vi "Update MC Listbox vColumn headers.vi"(0 "Multicolumn Listbox Ref":refnum<vi>, 1 "Interpret as Unicode (T)":bool=TRUE, 5 "Column Headers[]":string[](array[string]), 7 "Row Headers[]":string[](array[string]), 11 "Error in":errorcluster) -> (4 "Multicolumn Listbox Ref":refnum<vi>, 15 "error out":errorcluster)   [LabVIEW 2019, in "Language Selection.lvlib"]
doc: "Uses \"Column Header[]\" and \"Row Headers[]\" input arrays to translate a headers of a MulticolumnListbox control.\n- - -\nCopyright (c) 2026, Merecs Engineering GmbH"
uses:
  Language Selection.lvlib
panel:
  # "Connector Pane"
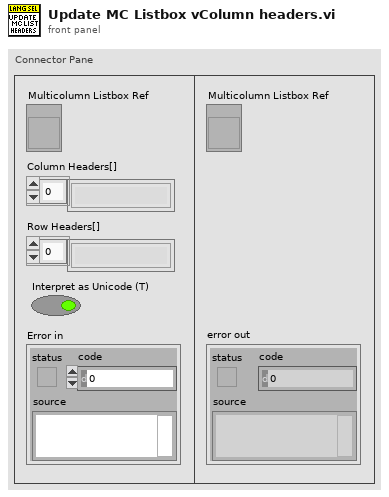
[diagram p1: front panel]
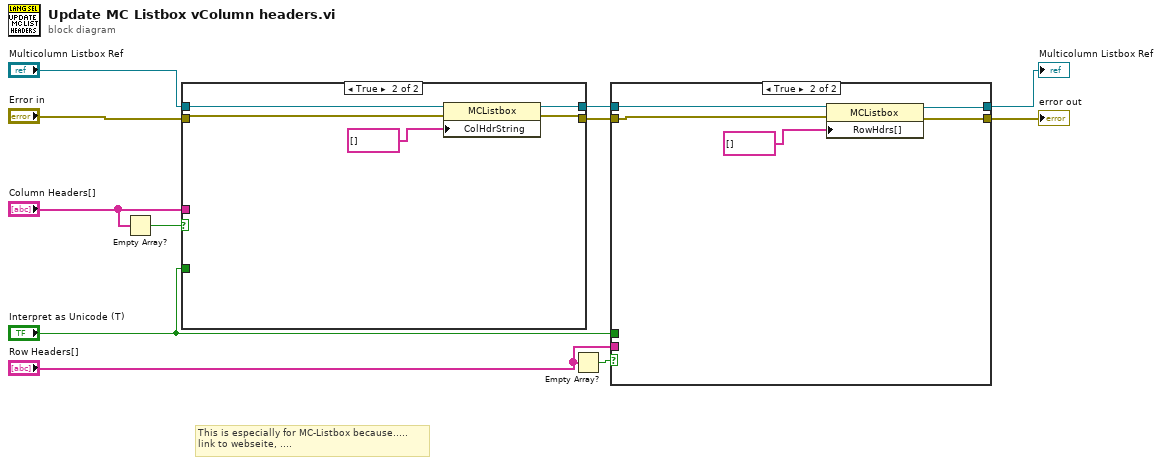
[diagram p0: block diagram]
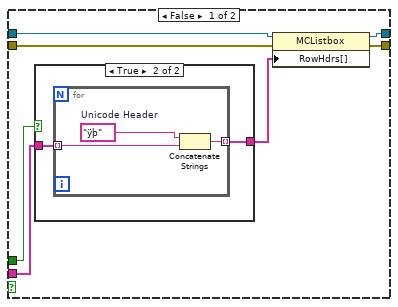
[diagram p2: hidden frame]
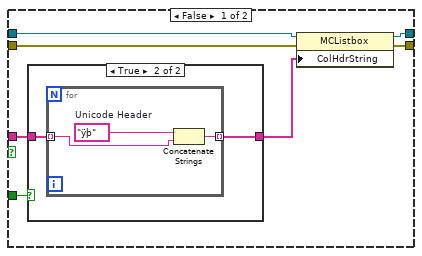
[diagram p4: hidden frame]
diagram:
  # "This is especially for MC-Listbox because.....\nlink to webseite, ...."
  n1 = Empty Array?(array="Column Headers[]") -> (empty?=w9:bool)
  n2 = case shown="True" w9 {
    tunnel: "Column Headers[]" -> [w18 _]
    tunnel: [w17 w29] -> w4
    tunnel: "Error in" -> [w15 w26]
    tunnel: "Multicolumn Listbox Ref" -> [w14 w27]
    tunnel: "Interpret as Unicode (T)" -> [w13 _]
    tunnel: [w12 w28] -> w7
    frame False {
      n3 = case shown="True" w13 {
        tunnel: w18 -> [w19 w21]
        tunnel: [w19 w20] -> w16
        frame False {
        }
        frame True {
          n4 = for {
            tunnel: w21 -> [w24] mode=indexing
            tunnel: [w23] -> w20 mode=indexing
            w22 = "ÿþ"  # Unicode Header
            n5 = Concatenate Strings(w22, w24) -> (w23:string)
          }
        }
      }
      n6 = property class="MCListbox"(reference=w14, error in=w15, "ColHdrString"=w16) -> (reference out=w12:refnum<vi>, error out=w17:errorcluster)
    }
    frame True {
      n7 = property class="MCListbox"(reference=w27, error in=w26, "ColHdrString"=string[] []) -> (reference out=w28:refnum<vi>, error out=w29:errorcluster)
    }
  }
  n8 = Empty Array?(array="Row Headers[]") -> (empty?=w3:bool)
  n9 = case shown="True" w3 {
    tunnel: "Row Headers[]" -> [w36 _]
    tunnel: [w35 w46] -> w6
    tunnel: w4 -> [w33 w45]
    tunnel: w7 -> [w32 w44]
    tunnel: "Interpret as Unicode (T)" -> [w31 _]
    tunnel: [w30 w47] -> w5
    frame False {
      n10 = case shown="True" w31 {
        tunnel: w36 -> [w37 w39]
        tunnel: [w37 w38] -> w34
        frame False {
        }
        frame True {
          n11 = for {
            tunnel: w39 -> [w42] mode=indexing
            tunnel: [w41] -> w38 mode=indexing
            w40 = "ÿþ"  # Unicode Header
            n12 = Concatenate Strings(w40, w42) -> (w41:string)
          }
        }
      }
      n13 = property class="MCListbox"(reference=w32, error in=w33, "RowHdrs[]"=w34) -> (reference out=w30:refnum<vi>, error out=w35:errorcluster)
    }
    frame True {
      n14 = property class="MCListbox"(reference=w44, error in=w45, "RowHdrs[]"=string[] []) -> (reference out=w47:refnum<vi>, error out=w46:errorcluster)
    }
  }
  "Multicolumn Listbox Ref" <- w5
  "error out" <- w6
